vi "m2 to m3.vi"   [LabVIEW 2017]
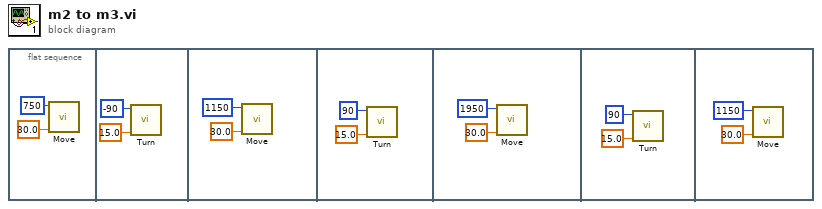
[diagram p0: block diagram]
diagram:
  n1 = flat-sequence {
    frame #0 {
      n2 = call "Move.vi"("Speed (0-30)"=30.0, "Distance (mm)"=750) -> ()  [unwired: 8 in]
    }
    frame #1 {
      n3 = call "Turn.vi"("Speed (0-30)"=15.0, "Angle (degrees)"=-90) -> ()  [unwired: 10 in]
    }
    frame #2 {
      n4 = call "Move.vi"("Speed (0-30)"=30.0, "Distance (mm)"=1150) -> ()  [unwired: 8 in]
    }
    frame #3 {
      n5 = call "Turn.vi"("Speed (0-30)"=15.0, "Angle (degrees)"=90) -> ()  [unwired: 10 in]
    }
    frame #4 {
      n6 = call "Move.vi"("Speed (0-30)"=30.0, "Distance (mm)"=1950) -> ()  [unwired: 8 in]
    }
    frame #5 {
      n7 = call "Turn.vi"("Speed (0-30)"=15.0, "Angle (degrees)"=90) -> ()  [unwired: 10 in]
    }
    frame #6 {
      n8 = call "Move.vi"("Speed (0-30)"=30.0, "Distance (mm)"=1150) -> ()  [unwired: 8 in]
    }
  }
